vi "libssh2_channel_receive_window_adjust2.vi"(8 "error in (no error)":errorcluster, 9 "force (F)":bool, 10 "adjustment":u32, 11 "channel":T1) -> (0 "error out":errorcluster, 2 "window":u32)   [LabVIEW 2017, in "libssh2.lvlib"]
doc: "Adjust the receive window for a channel by <B>adjustment</B> bytes.\nIf the amount to be adjusted is less than 1024 and <B>force</B> is zero the adjustment amount will be queued for a later packet.\n\nReturns the new size of the receive window."
uses:
  libssh2.lvlib
  Channel Refnum.ctl
  Acquire Session.vi
  Release Session.vi
  Not A Channel.vi
  <vilib>/Utility/error.llb/Error Cluster From Error Code.vi
  Global Settings.vi
  Read Channel Refnum.vi
  Read Session Refnum.vi
  <vilib>/Utility/semaphor.llb/Acquire Semaphore.vi
  <vilib>/Utility/semaphor.llb/Release Semaphore.vi
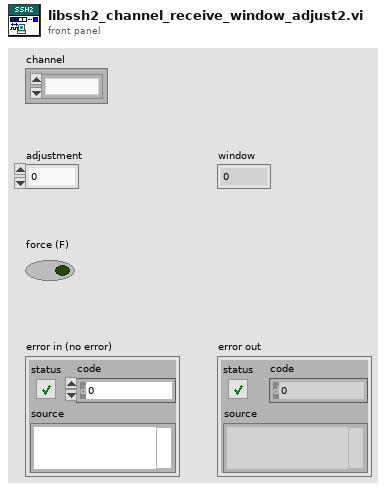
[diagram p1: front panel]
types:
  T1 = typedef "libssh2.lvlib/Channel Refnum.ctl" = refnum<k1>
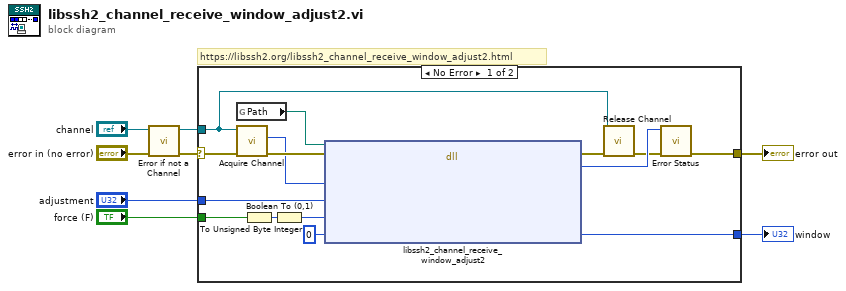
[diagram p0: block diagram]
diagram:
  # "https://libssh2.org/libssh2_channel_receive_window_adjust2.html"
  n1 = call "Error if not a Channel.vi"("error in (no error)"="error in (no error)", "channel"="channel") -> ("error out"=w6:errorcluster, "channel out"=w4:T1)  [unwired: 8 in]
  n2 = case shown="No Error" w6 {
    selector: w6 -> [w23 w24]
    tunnel: [w22 w24] -> w8
    tunnel: w4 -> [w9 _]
    tunnel: "adjustment" -> [w16 _]
    tunnel: "force (F)" -> [w15 _]
    tunnel: [w12 _] -> w1
    frame No Error {
      n3 = global read "Global Settings.vi" "Path"() -> (w18:path)
      n4 = call "Acquire Channel.vi"("error in (no error)"=w23, "channel"=w9) -> ("error out"=w20:errorcluster, "LIBSSH2_CHANNEL*"=w19:u64)  [unwired: 8 in]
      n5 = Boolean To (0,1)(Boolean=w15) -> (0, 1=w14:i16)
      n6 = To Unsigned Byte Integer(number=w14) -> (unsigned 8bit integer=w13:u8)
      n7 = dll-call lib="?" fn="libssh2_channel_receive_window_adjust2"(path in=w18, error in=w20, "channel"=w19, "adjustment"=w16, "force"=w13, "window"=u32 0) -> (error out=w21:errorcluster, "return value"=w17:i32, "window"=w12:u32)  [unwired: 4 in, 1 out]
      n8 = call "Release Channel.vi"("error in (no error)"=w21, "channel"=w9) -> ("error out"=w10:errorcluster)  [unwired: 9 in]
      n9 = call "Error Status.vi"("error in (no error)"=w10, "return value"=w17) -> ("error out"=w22:errorcluster)  [unwired: 8 in, 1 out]
    }
    frame Error {
    }
  }
  "error out" <- w8
  "window" <- w1
